vi "TEST - Wait Until Next ms Multiple.vi"(8 "error in (no error)":errorcluster) -> (0 "error out":errorcluster, 2 "pass":bool)   [LabVIEW 2020]
uses:
  <vilib>/addons/_JKI Toolkits/Caraya/classes/Assert/Assert True.vi
  source/library/openg_time.lvlib
  <vilib>/addons/_JKI Toolkits/Caraya/classes/Test/Test.lvclass
  <vilib>/addons/_JKI Toolkits/Caraya/classes/Assert/Assert.lvclass
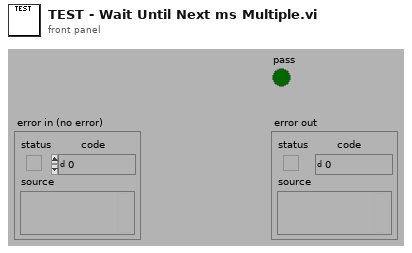
[diagram p1: front panel]
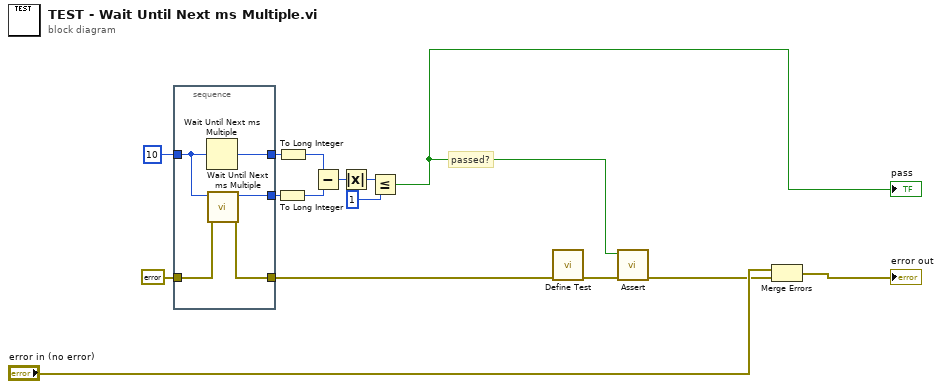
[diagram p0: block diagram]
diagram:
  # "passed?"
  n1 = stacked-sequence {
    tunnel: [w19] -> w2
    tunnel: errorcluster {"status"=FALSE, "code"=0, "source"=""} ("error in (no error)") -> [w20]
    tunnel: [w17] -> w11
    tunnel: u32 10 ("milliseconds to wait") -> [w18]
    tunnel: [w16] -> w12
    frame #0 {
      n2 = Wait Until Next ms Multiple(millisecond multiple=w18) -> (millisecond timer value=w16:u32)
      n3 = call "Wait Until Next ms Multiple.vi"("error in (no error)"=w20, "milliseconds to wait"=w18) -> ("error out"=w19:errorcluster, "millisecond timer value"=w17:u32)  [unwired: 8 in]
    }
  }
  n4 = To Long Integer(number=w11) -> (32bit integer=w8:i32)
  n5 = To Long Integer(number=w12) -> (32bit integer=w9:i32)
  n6 = Subtract(x=w9, y=w8) -> (x-y=w14:i32)
  n7 = Absolute Value(x=w14) -> (abs(x)=w10:i32)
  n8 = Less Or Equal?(x=w10, y=1) -> (x <= y?=w3:bool)
  "pass" <- w3
  n9 = call <vilib>:"Define Test.vi"("error in (no error)"=w2) -> ("error out"=w6:errorcluster)  [unwired: 9 in, 1 out]
  n10 = call-poly <vilib>:"Assert.vi"("error in (no error)"=w6, "True?"=w3) -> ("error out"=w1:errorcluster)  [unwired: 8 in, 1 out]
  n11 = Merge Errors("error in (no error)", w1) -> (→"error out":errorcluster)
